vi "Get Directory Icon.vi"(8 "error in":errorcluster, 11 "Directory Path":path) -> (0 "error out":errorcluster, 2 "Icon":picture, 3 "dup Directory Path":path)   [LabVIEW 2014, in "VIHelpeksAPI.lvlib"]
doc: "::: VI Helpeks :::\nCopyright (c) 2000-2026 Konstantin Shifershteyn. All rights reserved."
uses:
  VIHelpeksAPI.lvlib
panel:
  # "VI Helpeks\nCopyright (c) 2012-2026 Konstantin Shifershteyn"
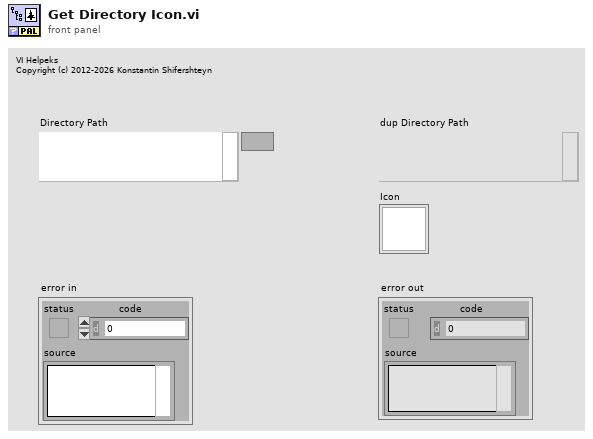
[diagram p1: front panel]
types:
  T1 = typedef "imagedata.ctl" = cluster{"image type":i32, "image depth":i32, "image":u8[], "mask":u8[], "colors":u32[], "Rectangle":cluster{"left":i16, "top":i16, "right":i16, "bottom":i16}}
  T2 = cluster{"left":i16, "top":i16, "right":i16, "bottom":i16}
  T3 = enum16{"User-specified Font", "Application Font", "System Font", "Dialog Font"}
  T4 = cluster{"Font Name:":string, "Size":i16, "Strikeout?":bool, "Italic?":bool, "Underline?":bool, "Outline?":bool, "Shadow?":bool, "Bold?":bool}
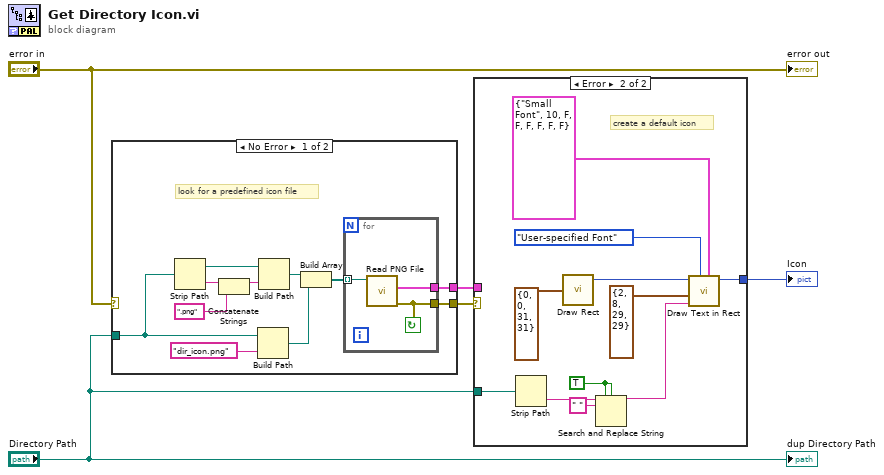
[diagram p0: block diagram]
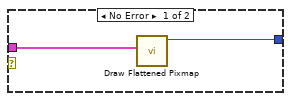
[diagram p3: hidden frame]
diagram:
  n1 = case shown="No Error" "error in" {
    selector: "error in" -> [_ w20]
    tunnel: [w8 w20] -> w5
    tunnel: [w7 _] -> w4
    tunnel: "Directory Path" -> [w6 _]
    frame No Error {
      # "look for a predefined icon file"
      n2 = Strip Path(path=w6) -> (stripped path=w14:path, name=w16:string)
      n3 = Concatenate Strings(w16, ".png") -> (w13:string)
      n4 = Build Path(base path=w6, name or relative path="dir_icon.png") -> (appended path=w10:path)
      n5 = Build Path(base path=w14, name or relative path=w13) -> (appended path=w11:path)
      n6 = Build Array(w11, w10) -> (w9:path[])
      n7 = for {
        tunnel: w9 -> [w19] mode=indexing
        tunnel: [w18] -> w8
        tunnel: [w17] -> w7
        stop <- w18 continue-if-true
        n8 = call <vilib>:"Read PNG File.vi"("path to PNG file"=w19) -> ("error out"=w18:errorcluster, "image data"=w17:T1)  [unwired: 8 in, 1 out]
      }
    }
    frame Error {
    }
  }
  n9 = case shown="Error" w5 {
    tunnel: w4 -> [w22 _]
    tunnel: [w21 w28] -> w3
    tunnel: "Directory Path" -> [_ w27]
    frame No Error {
      n10 = call <vilib>:"Draw Flattened Pixmap.vi"("image data"=w22) -> ("new picture"=w21:picture)  [unwired: 8 in]
    }
    frame Error {
      w24 = TRUE
      # "create a default icon"
      n11 = Strip Path(path=w27) -> (name=w26:string)  [unwired: 1 out]
      n12 = call <vilib>:"Draw Rect.vi"("rect"=T2 {"left"=0, "top"=0, "right"=31, "bottom"=31}) -> ("new picture"=w33:picture)  [unwired: 8 in]
      n13 = Search and Replace String(replace all?=w24, case sensitive?=w24, input string=w26, search string=" ") -> (result string=w23:string)  [unwired: 4 in, 3 out]
      n14 = call <vilib>:"Draw Text in Rect.vi"("[user-specified font]"=T4 {"Font Name:"="Small Font", "Size"=10, "Strikeout?"=FALSE, "Italic?"=FALSE, "Underline?"=FALSE, "Outline?"=FALSE, "Shadow?"=FALSE, "Bold?"=FALSE}, "desired font(Application)"=T3."User-specified Font", "text"=w23, "rect"=T2 {"left"=2, "top"=8, "right"=29, "bottom"=29}, "picture"=w33) -> ("new picture"=w28:picture)  [unwired: 6 in]
    }
  }
  "Icon" <- w3
  "error out" <- "error in"
  "dup Directory Path" <- "Directory Path"
